vi "Remove Session (byMailbox).vi"(8 "error in (no error)":errorcluster, 10 "SessionMailbox":refnum<queue>, 11 "MQTT Server":refnum<class "Server.lvclass">) -> (0 "error out":errorcluster, 3 "MQTT Server":refnum<class "Server.lvclass">)   [LabVIEW 2013, in "MQTT Server.lvlib" / "Server.lvclass"]
uses:
  Server.lvclass
  <vilib>/LabVIEW Open Source Project/MQTT Connection/MQTT_Base/Base Class/Response -- cluster.ctl
  <vilib>/LabVIEW Open Source Project/MQTT Control Packets/Control Packets/ControlPacket/ControlPacket.lvclass
  Server.lvclass/Server.ctl
  <vilib>/LabVIEW Open Source Project/MQTT Connection/MQTT_Base/Base Class/MQTT_Base.lvclass
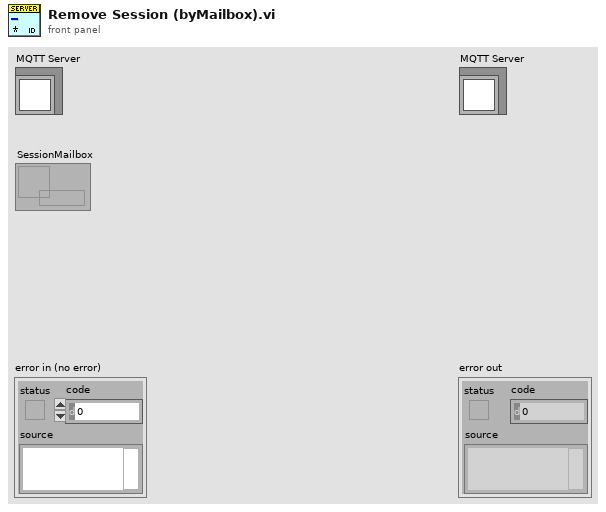
[diagram p1: front panel]
types:
  T1 = typedef "MQTT Server.lvlib/Server.lvclass/SessionRef -- cluster.ctl" = cluster{"ClientID":string, "SessionMailbox":refnum<queue>}
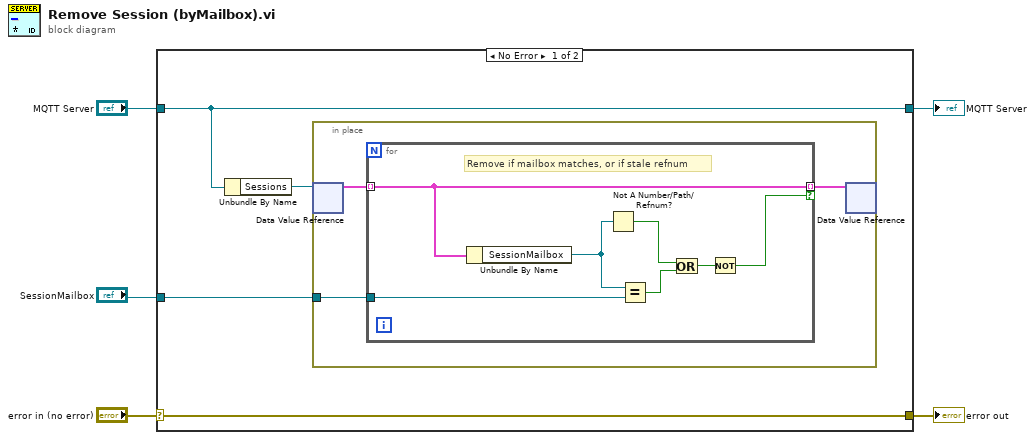
[diagram p0: block diagram]
diagram:
  n1 = case shown="No Error" "error in (no error)" {
    selector: "error in (no error)" -> [w6 w21]
    tunnel: [w6 w21] -> w4
    tunnel: [w8 w20] -> w2
    tunnel: "MQTT Server" -> [w8 w20]
    tunnel: "SessionMailbox" -> [w7 _]
    frame No Error {
      n2 = Unbundle By Name(w8) -> ("Sessions"=w9:refnum<data-value>)
      n3 = in-place {
        in-place-border: w7 -> [w12]
        n4 = in-place-dvr #1(w9) -> (w11:T1[])  [unwired: 1 out]
        n5 = for {
          tunnel: w12 -> [w17]
          tunnel: w11 -> [w19] mode=indexing
          tunnel: [w19] -> w10 mode=indexing if=w13
          # "Remove if mailbox matches, or if stale refnum"
          n6 = Unbundle By Name(w19) -> ("SessionMailbox"=w16:refnum<queue>)
          n7 = Not A Number/Path/Refnum?(number/path/refnum=w16) -> (NaN/Path/Refnum?=w18:bool)
          n8 = Equal?(x=w16, y=w17) -> (x = y?=w15:bool)
          n9 = Or(x=w18, y=w15) -> (x .or. y?=w14:bool)
          n10 = Not(x=w14) -> (.not. x?=w13:bool)
        }
        n11 = in-place-dvr #1(w10) -> ()  [unwired: 2 out]
      }
    }
    frame Error {
    }
  }
  "error out" <- w4
  "MQTT Server" <- w2
